vi "Globals.vi"() -> ()   [LabVIEW 2023, in "GettingStartedWindow.lvlib"]
uses:
  <resource>/modes/FRC/GSW/GettingStartedWindow.lvlib
panel:
  in  "error from reinit event creation":errorcluster
  in  "init buttons event":refnum<user-event>
  in  "error from close event creation":errorcluster
  in  "user event for close":refnum<user-event>
  in  "GSW Init Complete":bool
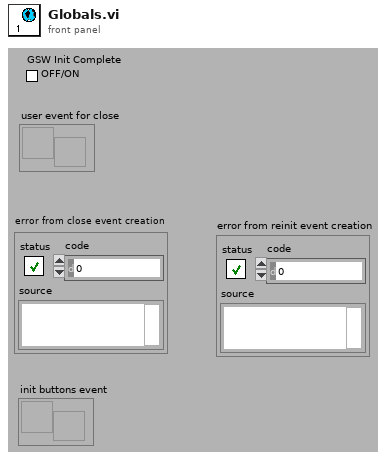
[diagram p1: front panel]
diagram:
